vi "Create Callback User Events.vi"(8 "error in":errorcluster, 11 "MyEventGrid in":refnum<class "MyEventGrid.lvclass">) -> (0 "error out":errorcluster, 3 "MyEventGrid out":refnum<class "MyEventGrid.lvclass">)   [LabVIEW 2026, in "MyEventGrid.lvclass"]
uses:
  MyEventGrid.lvclass
  source/Cells/Cell Context/Cell Context.lvclass
  MyEventGrid.lvclass/MyEventGrid.ctl
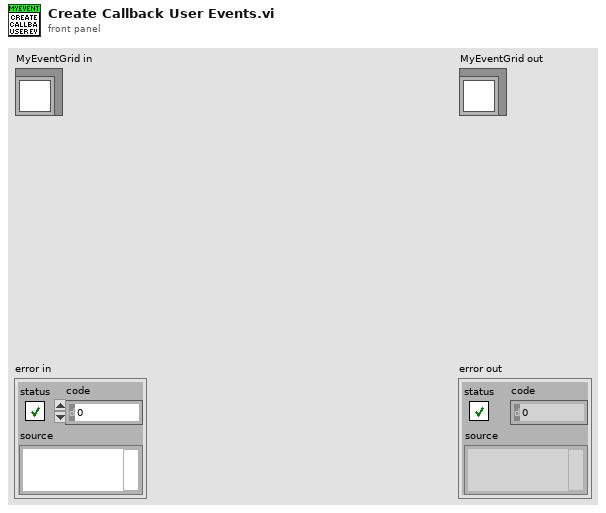
[diagram p1: front panel]
types:
  T1 = typedef "Rendezvous RefNum" = refnum<k1>
  T2 = cluster{"Context":refnum<class "Cell Context.lvclass">, "rendezvous":T1}
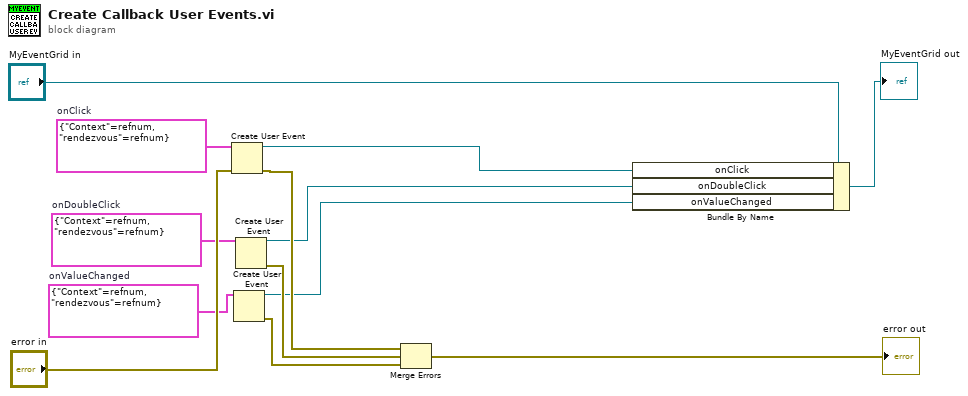
[diagram p0: block diagram]
diagram:
  w1 = T2 {"Context"=refnum, "rendezvous"=refnum}  # onDoubleClick
  w2 = T2 {"Context"=refnum, "rendezvous"=refnum}  # onValueChanged
  w3 = T2 {"Context"=refnum, "rendezvous"=refnum}  # onClick
  n1 = Create User Event(user event datatype=w3, error in="error in") -> (user event=w11:refnum<user-event>, error out=w8:errorcluster)
  n2 = Create User Event(user event datatype=w2) -> (user event=w5:refnum<user-event>, error out=w7:errorcluster)  [unwired: 1 in]
  n3 = Create User Event(user event datatype=w1) -> (user event=w6:refnum<user-event>, error out=w10:errorcluster)  [unwired: 1 in]
  n4 = Merge Errors(w8, w10, w7) -> (→"error out":errorcluster)
  n5 = Bundle By Name(cluster="MyEventGrid in", "onClick"=w11, "onDoubleClick"=w6, "onValueChanged"=w5) -> (→"MyEventGrid out":refnum<class "MyEventGrid.lvclass">)
